vi "libssh2_channel_forward_cancel.vi"(8 "error in (no error)":errorcluster, 11 "listener":T1) -> (0 "error out":errorcluster)   [LabVIEW 2017, in "libssh2.lvlib"]
doc: "Stop listening for inbound TCP connections on a listening channel."
uses:
  libssh2.lvlib
  Listener Refnum.ctl
  Global Settings.vi
  Read Session Refnum.vi
  <vilib>/Utility/semaphor.llb/Acquire Semaphore.vi
  <vilib>/Utility/semaphor.llb/Release Semaphore.vi
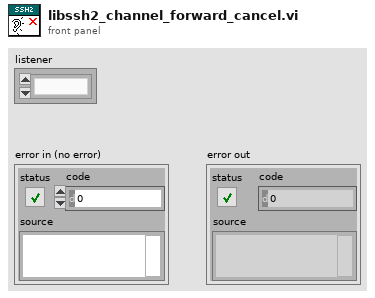
[diagram p1: front panel]
types:
  T1 = typedef "libssh2.lvlib/Listener Refnum.ctl" = refnum<k1>
  T2 = typedef "libssh2.lvlib/Session Refnum.ctl" = refnum<k1>
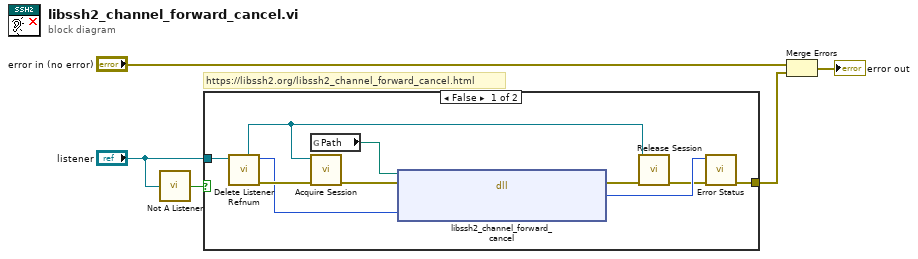
[diagram p0: block diagram]
diagram:
  # "https://libssh2.org/libssh2_channel_forward_cancel.html"
  n1 = call "Not A Listener.vi"("listener"="listener") -> ("Not a Listener?"=w1:bool)
  n2 = case shown="False" w1 {
    tunnel: "listener" -> [w14 _]
    tunnel: [w10 _] -> w3
    frame False {
      n3 = call "Delete Listener Refnum.vi"("listener"=w14) -> ("error out"=w15:errorcluster, "LIBSSH2_LISTENER*"=w13:u64, "session"=w6:T2)  [unwired: 8 in]
      n4 = global read "Global Settings.vi" "Path"() -> (w11:path)
      n5 = call "Acquire Session.vi"("error in (no error)"=w15, "session"=w6) -> ("error out"=w7:errorcluster)  [unwired: 7 in, 2 out]
      n6 = dll-call lib="?" fn="libssh2_channel_forward_cancel"(path in=w11, error in=w7, "listener"=w13) -> (error out=w12:errorcluster, "return value"=w9:i32)  [unwired: 2 in, 1 out]
      n7 = call "Release Session.vi"("error in (no error)"=w12, "session"=w6) -> ("error out"=w8:errorcluster)  [unwired: 9 in]
      n8 = call "Error Status.vi"("error in (no error)"=w8, "return value"=w9) -> ("error out"=w10:errorcluster)  [unwired: 8 in, 1 out]
    }
    frame True {
    }
  }
  n9 = Merge Errors("error in (no error)", w3) -> (→"error out":errorcluster)
